vi "VIH Utility - FILE - Get and Replace Extension (File Path).vi"(10 "new extension (none)":string, 11 "file path":path) -> (2 "extension":string, 3 "new file path":path)   [LabVIEW 2014]
doc: "::: VI Helpeks :::\nCopyright (c) 2000-2026 Konstantin Shifershteyn. All rights reserved."
panel:
  # "VI Helpeks\nCopyright (c) 2012-2026 Konstantin Shifershteyn"
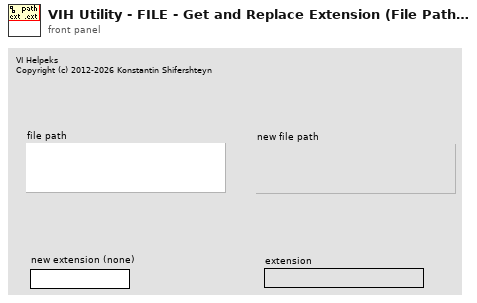
[diagram p1: front panel]
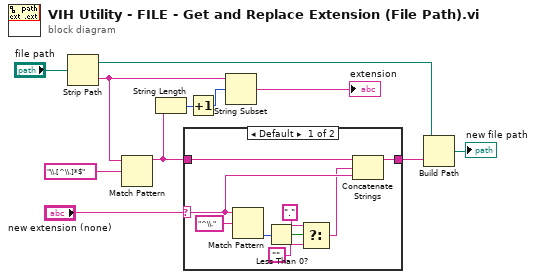
[diagram p0: block diagram]
diagram:
  n1 = Strip Path(path="file path") -> (stripped path=w7:path, name=w5:string)
  n2 = Match Pattern(string=w5, regular expression="\\.[^\\.]*$") -> (before substring=w2:string)  [unwired: 4 out]
  n3 = String Length(string=w2) -> (length=w3:i32)
  n4 = case shown="Default" "new extension (none)" {
    selector: "new extension (none)" -> [w18 _]
    tunnel: w2 -> [w19 w21]
    tunnel: [w12 w21] -> w8
    frame Default {
      n5 = Match Pattern(string=w18, regular expression="^\\.") -> (offset past match=w17:i32)  [unwired: 4 out]
      n6 = Less Than 0?(x=w17) -> (x < 0?=w16:bool)
      n7 = Select(t=".", s=w16, f="") -> (s? t:f=w13:string)
      n8 = Concatenate Strings(w19, w13, w18) -> (w12:string)
    }
    frame "" {
    }
  }
  n9 = Increment(x=w3) -> (x+1=w1:i32)
  n10 = String Subset(string=w5, offset (0)=w1) -> (substring=→"extension":string)  [unwired: 1 out]
  n11 = Build Path(base path=w7, name or relative path=w8) -> (appended path=→"new file path":path)
